vi "ParametricCurve.vi"(7 "LabVIEW Web Service Request":refnum<class "Web Request.lvclass">) -> ()   [LabVIEW 2016]
uses:
  <vilib>/wsapi/Web Request.lvclass
  <vilib>/Analysis/6fits.llb/Prediction Interval (Gauss).vi
  <vilib>/Analysis/NI_AALPro.lvlib
panel:
  # "Use the Web Service Request input terminal to call the VIs on the Web Services palette. Do not remove it from the connector pane unless you don't need access to the palette."
  # "Each additional control wired to the connector pane will be available as an input in the URL. To include an indicator in terminal-mode output (the default setting), it must also be wired to the connector pane."
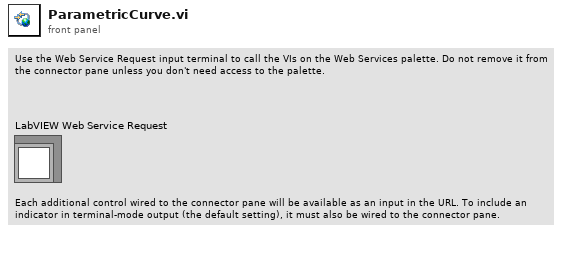
[diagram p1: front panel]
types:
  T1 = cluster{"X":dbl[], "Y":dbl[], "Best Gaussian Fit":dbl[], "Upper Bound":dbl[], "Lower Bound":dbl[]}
  T2 = enum16{"Linear", "Exponential", "Power", "Gaussian", "Logarithmic"}
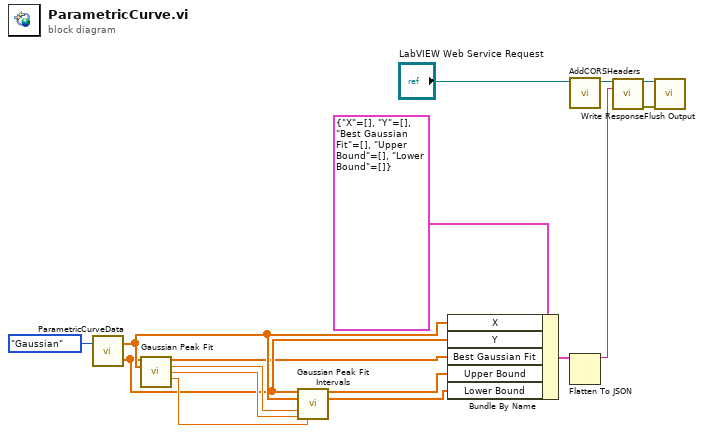
[diagram p0: block diagram]
diagram:
  n1 = call "ParametricCurveData.vi"("Signal type"=T2."Gaussian") -> ("Y"=w10:dbl[], "X"=w11:dbl[])  [unwired: 1 in]
  n2 = call <vilib>:"Gaussian Peak Fit.vi"("Y"=w10, "X"=w11) -> ("Best Gaussian Fit"=w9:dbl[], "amplitude"=w15:dbl, "center"=w14:dbl, "standard deviation"=w13:dbl)  [unwired: 7 in, 3 out]
  n3 = call-poly <vilib>:"Gaussian Peak Fit Intervals.vi"("Y"=w10, "X"=w11, "amplitude"=w15, "center"=w14, "standard deviation"=w13) -> ("Upper Bound"=w8:dbl[], "Lower Bound"=w7:dbl[])  [unwired: 8 in, 1 out]
  n4 = Bundle By Name(cluster=T1 {"X"=[], "Y"=[], "Best Gaussian Fit"=[], "Upper Bound"=[], "Lower Bound"=[]}, "X"=w11, "Y"=w10, "Best Gaussian Fit"=w9, "Upper Bound"=w8, "Lower Bound"=w7) -> (w12:T1)
  n5 = call "AddCORSHeaders.vi"("Web Request in"="LabVIEW Web Service Request") -> ("Web Request out"=w2:refnum<class "Web Request.lvclass">)  [unwired: 10 in]
  n6 = Flatten To JSON(anything=w12) -> (JSON string=w5:string)  [unwired: 2 in, 1 out]
  n7 = call <vilib>:"Write Response.vi"("LabVIEW Web Service Request"=w2, "response string"=w5) -> ("LabVIEW Web Service Request out"=w4:refnum<class "Web Request.lvclass">, "error out"=w3:errorcluster)  [unwired: 12 in]
  n8 = call <vilib>:"Flush Output.vi"("LabVIEW Web Service Request"=w4, "error in (no error)"=w3) -> ()  [unwired: 12 in, 2 out]
